vi "Get Registry Message Event.vi"() -> (3 "registry message event":refnum<user-event>)   [LabVIEW 2018, in "GLog.lvlib" / "Registry.lvlib"]
uses:
  Registry.lvlib
  Registry Message.ctl
  Registry Actions.ctl
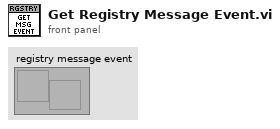
[diagram p1: front panel]
types:
  T1 = typedef "GLog.lvlib/Registry.lvlib/Registry Message.ctl" = cluster{"action":T2, "data":variant, "return notifier":refnum<notifier>}
  T2 = typedef "GLog.lvlib/Registry.lvlib/Registry Actions.ctl" = enum16{"Register", "Log", "Enable", "Enable All", "Disable", "Disable All", "Get Enable State", "Get Minimum Log Level", "Set Minimum Log Level", "Set All Minimum Log Level", "Get Logger Info", "Get All Logger Info", "List", "Unregister", "Unregister All", "Shutdown"}
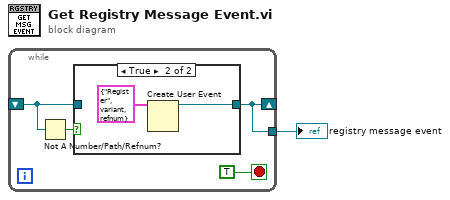
[diagram p0: block diagram]
diagram:
  n1 = while {
    tunnel: [w5] -> w1
    shift-right: [w5] -> _
    shift-left: _ -> [w3]
    stop <- TRUE stop-if-true
    n2 = Not A Number/Path/Refnum?(number/path/refnum=w3) -> (NaN/Path/Refnum?=w2:bool)
    n3 = case shown="True" w2 {
      tunnel: [w6 w8] -> w5
      tunnel: w3 -> [w6 _]
      frame False {
      }
      frame True {
        n4 = Create User Event(user event datatype=T1 {"action"=enum."Register", "data"=variant, "return notifier"=refnum} ("registry message")) -> (user event=w8:refnum<user-event>)  [unwired: 1 in, 1 out]
      }
    }
  }
  "registry message event" <- w1
